vi "Translate gRPC Method FullName.vi"(8 "error in (no error)":errorcluster, 11 "Method Full Name in":string) -> (0 "error out":errorcluster, 3 "Method Full Name out":string)   [LabVIEW 2019, in "gRPC Template Creation Utility.lvlib"]
uses:
  gRPC Template Creation Utility.lvlib
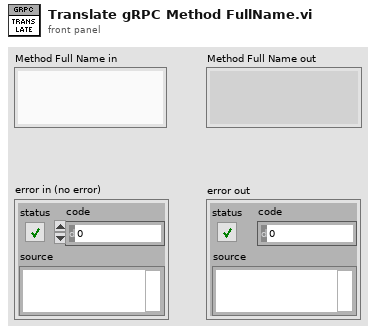
[diagram p1: front panel]
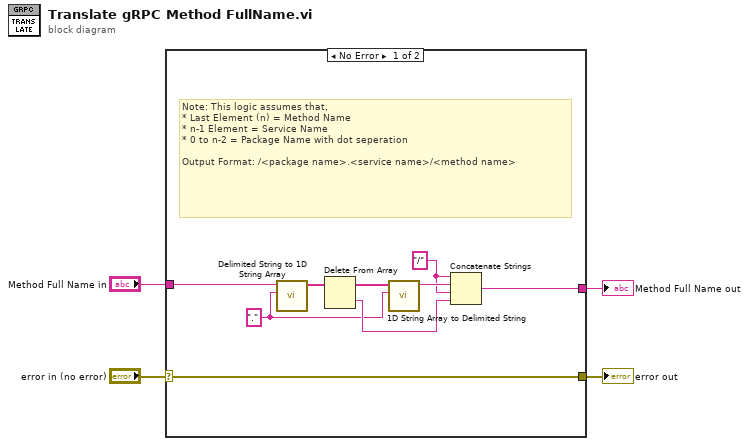
[diagram p0: block diagram]
diagram:
  n1 = case shown="No Error" "error in (no error)" {
    selector: "error in (no error)" -> [w11 w15]
    tunnel: [w10 w14] -> w4
    tunnel: "Method Full Name in" -> [w12 w14]
    tunnel: [w11 w15] -> w1
    frame No Error {
      w7 = "/"
      w5 = "." ("delimiter")
      # "Note: This logic assumes that,\n* Last Element (n) = Method Name\n* n-1 Element = Service Name\n* 0 to n-2 = Package Name with dot seperation\n\nOutput Format: /<package name>.<service name>/<method name>"
      n2 = call <vilib>:"Delimited String to 1D String Array.vi"("delimiter"=w5, "delimited string"=w12) -> ("string array"=w13:string[])  [unwired: 9 in]
      n3 = Delete From Array(array=w13) -> (deleted portion=w6:string, array with subset deleted=w9:string[])  [unwired: 2 in]
      n4 = call <vilib>:"1D String Array to Delimited String.vi"("delimiter"=w5, "string array"=w9) -> ("delimited string"=w8:string)  [unwired: 9 in]
      n5 = Concatenate Strings(w7, w8, w7, w6) -> (w10:string)
    }
    frame Error {
    }
  }
  "Method Full Name out" <- w4
  "error out" <- w1
